vi "Cut Half Data.vi"(8 "error in (no error)":errorcluster caption="错误输入（无错误）", 11 "Data Viewer 输入":refnum<class "Data Viewer.lvclass">) -> (0 "error out":errorcluster caption="错误输出", 3 "Data Viewer 输出":refnum<class "Data Viewer.lvclass">)   [LabVIEW 2020, in "Data Viewer.lvlib" / "Data Viewer.lvclass"]
uses:
  Data Viewer.lvclass
  Data Viewer.lvclass/Data Viewer.ctl
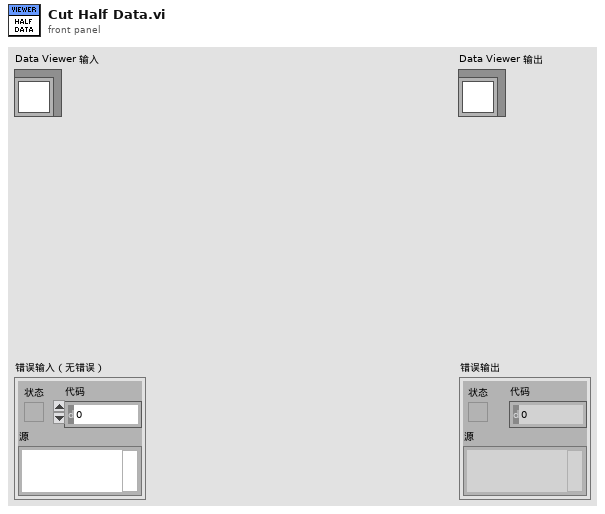
[diagram p1: front panel]
types:
  T1 = typedef "Data Viewer.lvlib/Data Serie--cluster.ctl" = cluster{"Name":string, "Unit":string, "Sample Rate[Hz]":dbl, "Delta t[S]":dbl, "t0":timestamp, "Length":i32, "Time":timestamp[], "Value":dbl[]}
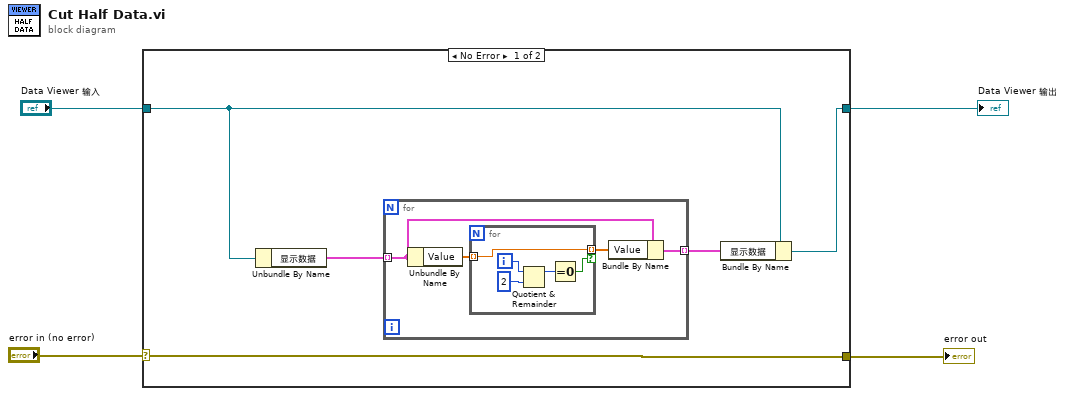
[diagram p0: block diagram]
diagram:
  n1 = case shown="No Error" "error in (no error)" {
    selector: "error in (no error)" -> [w9 w20]
    tunnel: [w9 w20] -> w3
    tunnel: [w6 w19] -> w1
    tunnel: "Data Viewer 输入" -> [w8 w19]
    frame No Error {
      n2 = Unbundle By Name(w8) -> ("显示数据"=w7:T1[])
      n3 = for {
        tunnel: w7 -> [w12] mode=indexing
        tunnel: [w10] -> w5 mode=indexing
        n4 = Unbundle By Name(w12) -> ("Value"=w13:dbl[])
        n5 = for {
          tunnel: w13 -> [w16] mode=indexing
          tunnel: [w16] -> w11 mode=indexing if=w15
          i -> [w17]
          n6 = Quotient & Remainder(x=w17, y=2) -> (x-y*floor(x/y)=w14:i32)  [unwired: 1 out]
          n7 = Equal To 0?(x=w14) -> (x = 0?=w15:bool)
        }
        n8 = Bundle By Name(cluster=w12, "Value"=w11) -> (w10:T1)
      }
      n9 = Bundle By Name(cluster=w8, "显示数据"=w5) -> (w6:refnum<class "Data Viewer.lvclass">)
    }
    frame Error {
    }
  }
  "error out" <- w3
  "Data Viewer 输出" <- w1
